vi "Audio_Close.vi"(0 "Task ID":u32, 11 "error in":errorcluster) -> (15 "error out":errorcluster)   [LabVIEW 2020, in "GH_App.lvlib"]
doc: "Closes the sound channel after the audio loop has ended (error in = error of the audio loop; the error of the released sound queue is normal there)."
uses:
  GH_App.lvlib
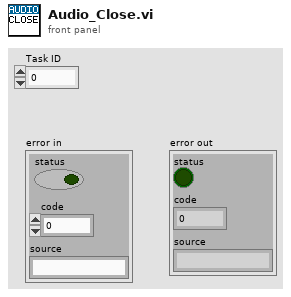
[diagram p1: front panel]
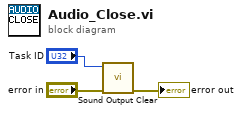
[diagram p0: block diagram]
diagram:
  n1 = call <vilib>:"Sound Output Clear.vi"("error in (no error)"="error in", "task ID"="Task ID") -> ("error out"=→"error out":errorcluster)  [unwired: 9 in]
